vi "Torque Test.vi"(6 "wait for reply (T)":bool=TRUE, 7 "On Time [ms]":dbl, 8 "error in":errorcluster, 9 "Speed [rpm]":T3=9.818181818181818 min=0.0 max=100.0 scale=0.0..100.0, 10 "Array 2":T4, 11 "Module ID":i32=-1) -> (0 "error out":errorcluster, 1 "timed out?":bool, 2 "Array 3":T1, 5 "Complete?":bool)   [LabVIEW 2025, in "Sequencer.lvlib"]
doc: "_____\nCreated using DQMH Framework: Event Scripter 7.1.2.1547."
uses:
  Sequencer.lvlib
  Controls/Motor Speed Slider.ctl
  Controls/Sequencer/step cluster.ctl
  Controls/Sequencer/sequence array.ctl
  Torque Test Argument--cluster.ctl
  Controls/Sequencer/results cluster.ctl
  Controls/Sequencer/results array.ctl
  Torque Test (Reply Payload)--cluster.ctl
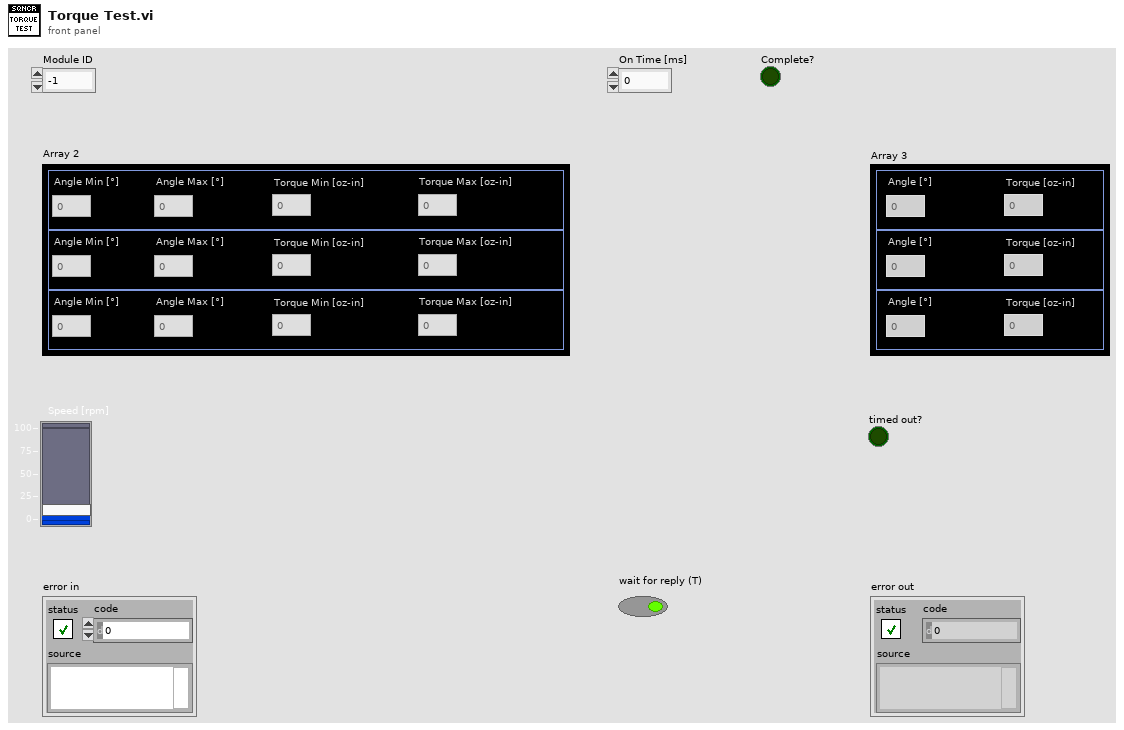
[diagram p1: front panel]
types:
  T1 = typedef "results array.ctl" = T2[]
  T2 = typedef "results cluster.ctl" = cluster{"Angle [°]":dbl, "Torque [oz-in]":dbl}
  T3 = typedef "Motor Speed Slider.ctl" = dbl
  T4 = typedef "sequence array.ctl" = T5[]
  T5 = typedef "step cluster.ctl" = cluster{"Angle Min [°]":dbl, "Angle Max [°]":dbl, "Torque Min [oz-in]":dbl, "Torque Max [oz-in]":dbl}
  T6 = typedef "Sequencer.lvlib/Torque Test Argument--cluster.ctl" = cluster{"Module ID":i32, "Array 2":T4, "Speed [rpm]":T3, "On Time [ms]":dbl, "Wait Notifier":refnum<notifier>, "wait for reply":bool}
  T7 = typedef "Sequencer.lvlib/Request Events--cluster.ctl" = cluster{"Stop Module":refnum<user-event>, "Show Panel":refnum<user-event>, "Hide Panel":refnum<user-event>, "Show Diagram":refnum<user-event>, "Get Module Execution Status":refnum<user-event>, "Get Modules":refnum<user-event>, "Home":refnum<user-event>, "Home Stepper":refnum<user-event>, "Go To Angle":refnum<user-event>, "Part Removal Position":refnum<user-event>, "Torque Test":refnum<user-event>}
  T8 = typedef "Sequencer.lvlib/Torque Test (Reply Payload)--cluster.ctl" = cluster{"Module ID":i32, "Array 2":T1, "Complete?":bool, "error":errorcluster}
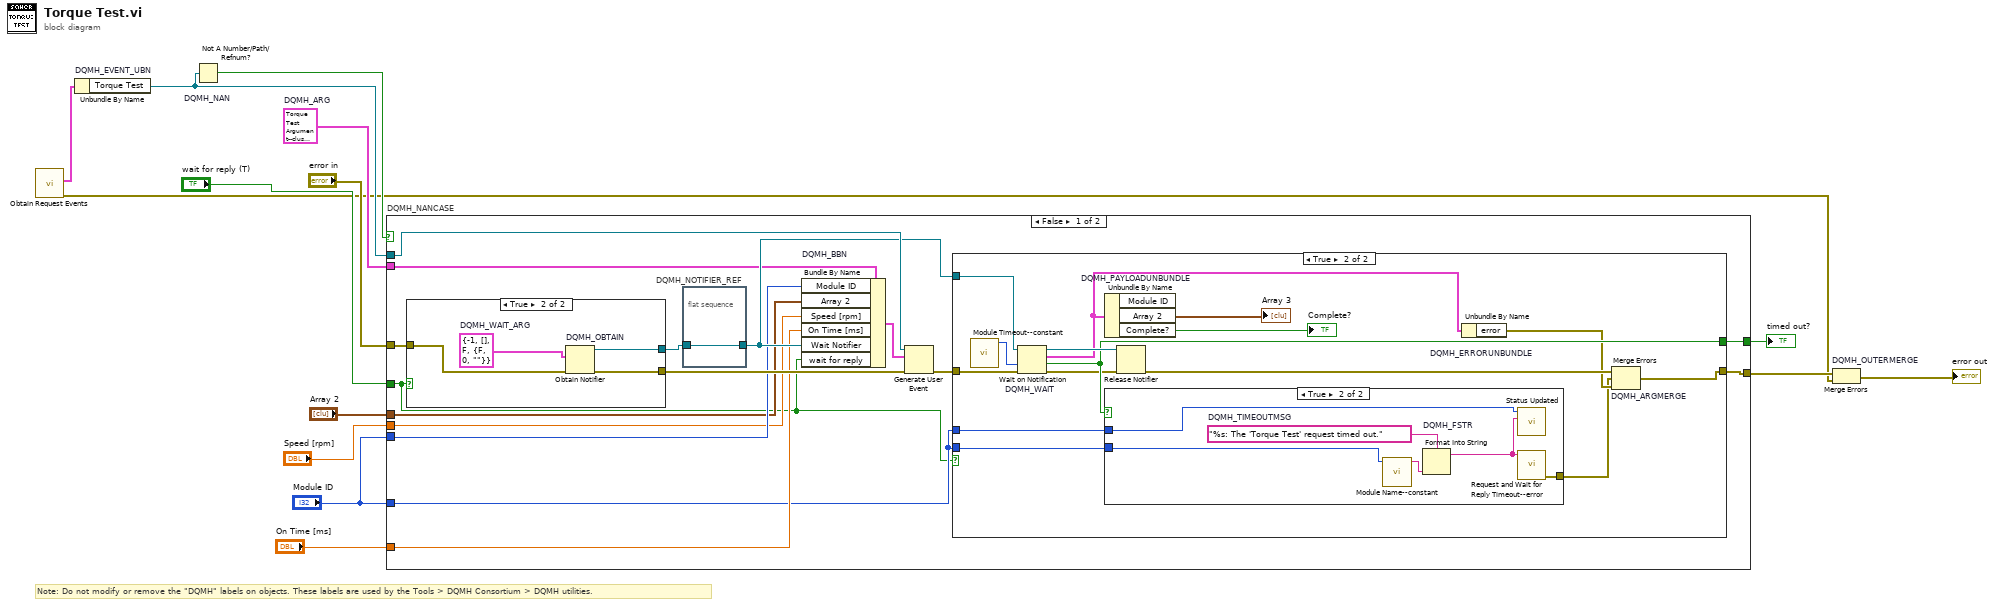
[diagram p0: block diagram]
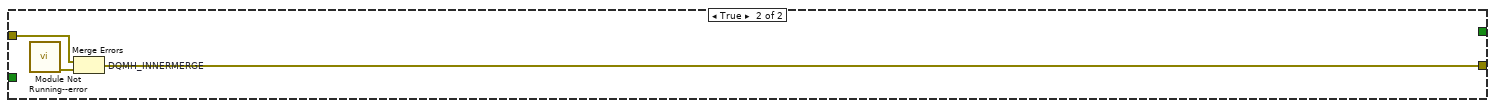
[diagram p5: hidden frame]
diagram:
  w8 = T6 {"Module ID"=-1, "Array 2"=[], "Speed [rpm]"=9.818181818181818, "On Time [ms]"=0.0, "Wait Notifier"=refnum, "wait for reply"=FALSE}  # DQMH_ARG
  # "Note: Do not modify or remove the \"DQMH\" labels on objects. These labels are used by the Tools > DQMH Consortium > DQMH utilities."
  n1 = call "Obtain Request Events.vi"() -> ("error out"=w2:errorcluster, "Sequencer Request Events"=w1:T7)  [unwired: 10 in]
  n2 = Unbundle By Name "DQMH_EVENT_UBN"(w1) -> ("Torque Test"=w12:refnum<user-event>)
  n3 = Not A Number/Path/Refnum? "DQMH_NAN"(number/path/refnum=w12) -> (NaN/Path/Refnum?=w11:bool)
  n4 = case "DQMH_NANCASE" shown="False" w11 {
    tunnel: "error in" -> [w30 w61]
    tunnel: w12 -> [w28 _]
    tunnel: [w25 w60] -> w9
    tunnel: [w26 _] -> w10
    tunnel: w8 -> [w21 _]
    tunnel: "Module ID" -> [w20 _]
    tunnel: "Array 2" -> [w19 _]
    tunnel: "Speed [rpm]" -> [w18 _]
    tunnel: "On Time [ms]" -> [w17 _]
    tunnel: "Module ID" -> [w16 _]
    tunnel: "wait for reply (T)" -> [w15 _]
    frame False {
      n5 = case shown="True" w15 {
        tunnel: w30 -> [w54 w58]
        tunnel: [w54 w57] -> w27
        tunnel: [_ w55] -> w23
        frame False {
        }
        frame True {
          w56 = T8 {"Module ID"=-1, "Array 2"=[], "Complete?"=FALSE, "error"={"status"=FALSE, "code"=0, "source"=""}}  # DQMH_WAIT_ARG
          n6 = Obtain Notifier "DQMH_OBTAIN"(notification data type=w56, error in (no error)=w58) -> (notifier out=w55:refnum<notifier>, error out=w57:errorcluster)  [unwired: 2 in, 1 out]
        }
      }
      n7 = flat-sequence "DQMH_NOTIFIER_REF" {
        tunnel: w23 -> [w31]
        tunnel: [w31] -> w22
        frame #0 {
        }
      }
      n8 = Bundle By Name "DQMH_BBN"(cluster=w21, "Module ID"=w20, "Array 2"=w19, "Speed [rpm]"=w18, "On Time [ms]"=w17, "Wait Notifier"=w22, "wait for reply"=w15) -> (w24:T6)
      n9 = Generate User Event(user event=w28, event data cluster=w24, error in=w27) -> (error out=w29:errorcluster)  [unwired: 1 in, 1 out]
      n10 = case shown="True" w15 {
        tunnel: w29 -> [w32 w47]
        tunnel: w22 -> [_ w46]
        tunnel: [_ w44] -> w26
        tunnel: [w32 w43] -> w25
        tunnel: w16 -> [_ w34]
        tunnel: w16 -> [_ w33]
        frame False {
        }
        frame True {
          n11 = call "Module Timeout--constant.vi"() -> ("Module Timeout"=w37:i32)  [unwired: 11 in]
          n12 = Wait on Notification "DQMH_WAIT"(notifier=w46, timeout in ms (-1)=w37, error in (no error)=w47) -> (notifier out=w45:refnum<notifier>, notification=w38:T8, timed out?=w44:bool, error out=w42:errorcluster)  [unwired: 1 in]
          n13 = Unbundle By Name "DQMH_PAYLOADUNBUNDLE"(w38) -> ("Array 2"=→"Array 3":T1, "Complete?"=→"Complete?":bool)  [unwired: 1 out]
          n14 = case shown="True" w44 {
            tunnel: [_ w51] -> w39
            tunnel: w34 -> [_ w49]
            tunnel: w33 -> [_ w48]
            frame False {
            }
            frame True {
              w53 = "%s: The 'Torque Test' request timed out."  # DQMH_TIMEOUTMSG
              n15 = call "Module Name--constant.vi"("Module ID"=w48) -> ("Module Name"=w50:string)  [unwired: 10 in]
              n16 = Format Into String "DQMH_FSTR"(format string=w53, w50) -> (resulting string=w52:string)  [unwired: 2 in, 1 out]
              n17 = call "Status Updated.vi"("Status"=w52, "Module ID"=w49) -> ()  [unwired: 9 in, 1 out]
              n18 = call "Request and Wait for Reply Timeout--error.vi"("Error Message"=w52) -> ("error out"=w51:errorcluster)  [unwired: 10 in]
            }
          }
          n19 = Release Notifier(notifier=w45, error in (no error)=w42) -> (error out=w41:errorcluster)  [unwired: 1 in, 2 out]
          n20 = Unbundle By Name "DQMH_ERRORUNBUNDLE"(w38) -> ("error"=w40:errorcluster)
          n21 = Merge Errors "DQMH_ARGMERGE"(w41, w39, w40) -> (w43:errorcluster)
        }
      }
    }
    frame True {
      n22 = call "Module Not Running--error.vi"() -> ("error out"=w59:errorcluster)  [unwired: 11 in]
      n23 = Merge Errors "DQMH_INNERMERGE"(w61, w59) -> (w60:errorcluster)
    }
  }
  "timed out?" <- w10
  n24 = Merge Errors "DQMH_OUTERMERGE"(w9, w2) -> (→"error out":errorcluster)
